vi "LinearSystemId_DiffDrv_ID_Pack_Model_Params.vi"(8 "Ka Angular":dbl, 9 "Kv Angular":dbl, 10 "Ka Linear":dbl, 11 "Kv Linear":dbl) -> (3 "DiffDrv_LinearSystem":T1)   [LabVIEW 2019, in "Trajectory_Library.lvlib"]
doc: "Creates a Differential Drive Train linear system from the drive train characterization (identification) data. \n\nThe linear system is define as:\n - states\n - left velocity (m/s)\n - right velocity (m/s)\n - inputs\n - left voltage (volts)\n - right voltage(volts)\n - outputs\n - left velocity (m/s)\n - right velocity (m/s)\n\nInputs:\n - Kv Linear -- double -- Linear velocity constant (volts/(meter/sec)\n - Ka Linear -- double -- Linear acceleration constant (volts/(meter/sec^2))\n - Kv Angular -- double -- Rotational velocity constant (volts/(meter/sec)\n - Ka Angular -- double -- Rotational acceleration constant (volts/(meter/sec^2))\n\nOutputs:\n - DiffDrive Linear Syste -- Linear System -- The resulting differential drive linear system."
uses:
  Trajectory_Library.lvlib
  <vilib>/Analysis/Matrix/Datatypes/RealMatrix.ctl
  <vilib>/Analysis/Matrix/NI_Matrix.lvlib
  TypeDef/LINEAR_SYSTEM.ctl
panel:
  # "<States,States>"
  # "<States,Inputs>"
  # "<Outputs,States>"
  # "<Outputs,Inputs>"
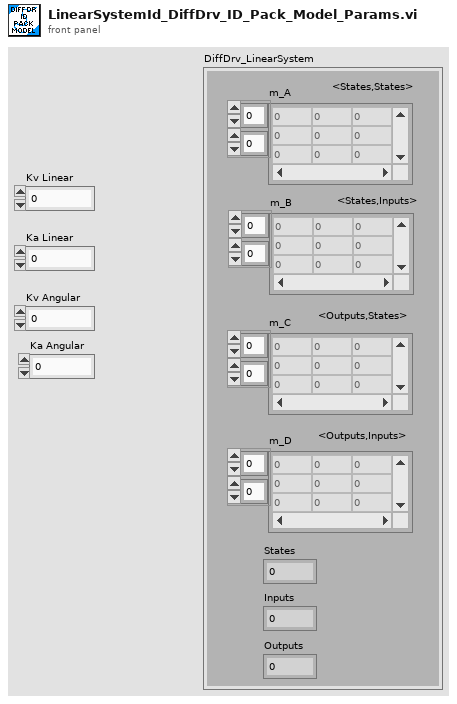
[diagram p1: front panel]
types:
  T1 = typedef "Trajectory_Library.lvlib/LINEAR_SYSTEM.ctl" = cluster{"m_A":T2, "m_B":T2, "m_C":T2, "m_D":T2, "States":i32, "Inputs":i32, "Outputs":i32}
  T2 = typedef "NI_Matrix.lvlib/RealMatrix.ctl" = dbl[][]
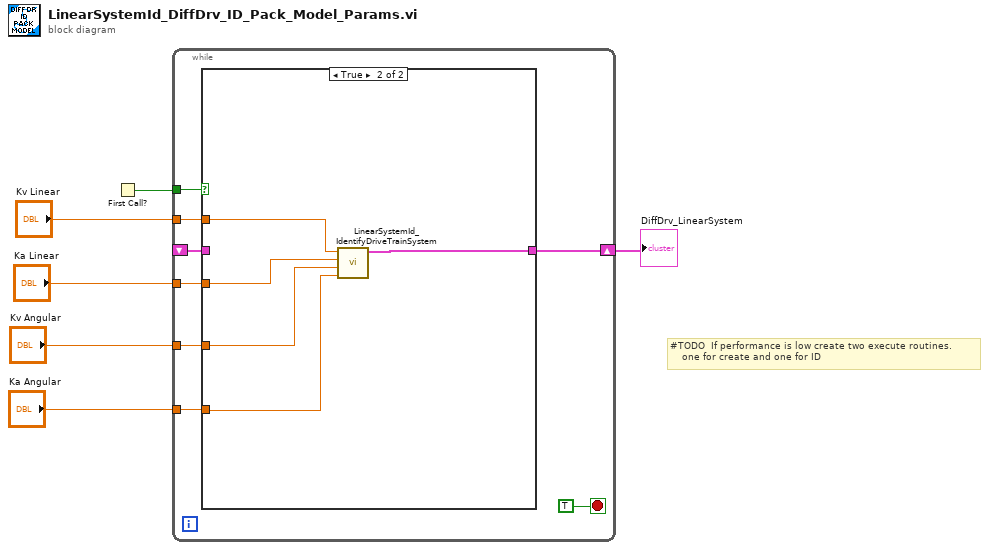
[diagram p0: block diagram]
diagram:
  # "#TODO  If performance is low create two execute routines.\n    one for create and one for ID"
  n1 = First Call?() -> (First Call?: T/F=w2:bool)
  n2 = while {
    tunnel: "Kv Linear" -> [w13]
    tunnel: "Ka Linear" -> [w12]
    tunnel: "Kv Angular" -> [w11]
    tunnel: "Ka Angular" -> [w10]
    shift-right: [w9] -> w1
    shift-left: _ -> [w7]
    tunnel: w2 -> [w8]
    stop <- TRUE stop-if-true
    n3 = case shown="True" w8 {
      tunnel: w13 -> [_ w20]
      tunnel: w12 -> [_ w19]
      tunnel: w11 -> [_ w18]
      tunnel: w10 -> [_ w17]
      tunnel: [w15 w16] -> w9
      tunnel: w7 -> [w15 _]
      frame False {
      }
      frame True {
        n4 = call "LinearSystemId_IdentifyDriveTrainSystem.vi"("kAAngular"=w17, "kVAngular"=w18, "kALinear"=w19, "kVLinear"=w20) -> ("Linearsystem"=w16:T1)  [unwired: 6 in, 1 out]
      }
    }
  }
  "DiffDrv_LinearSystem" <- w1
